vi "Get Local UTC Offset.vi"(9 "timestamp (now)":timestamp, 10 "UTC? (F)":bool) -> (1 "UTC Offset String":string, 2 "UTC Offset":T1=enum."UTC+00:00", 5 "UTC Offset (minutes)":i32, 7 "UTC Offset (hours)":i32)   [LabVIEW 2013]
uses:
  UTC Offsets -- enum.ctl
  <vilib>/regexp/Match Regular Expression.xnode
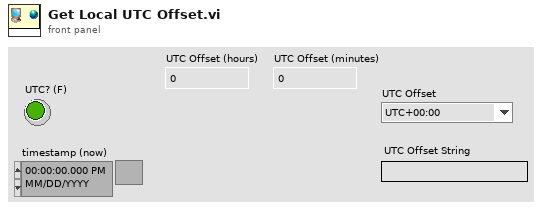
[diagram p1: front panel]
types:
  T1 = typedef "UTC Offsets -- enum.ctl" = enum16{"UTC-12:00", "UTC-11:00", "UTC-10:00", "UTC-09:30", "UTC-09:00", "UTC-08:00", "UTC-07:00", "UTC-06:00", "UTC-05:00", "UTC-04:00", "UTC-03:30", "UTC-03:00", "UTC-02:00", "UTC-01:00", "UTC-00:00", "UTC+00:00", "UTC+01:00", "UTC+02:00", "UTC+03:00", "UTC+03:30", "UTC+04:00", "UTC+04:30", "UTC+05:00", "UTC+05:30", "UTC+05:45", "UTC+06:00", "UTC+06:30", "UTC+07:00", "UTC+08:00", "UTC+08:45", "UTC+09:00", "UTC+09:30", "UTC+10:00", "UTC+10:30", "UTC+11:00", "UTC+12:00", "UTC+12:45", "UTC+13:00", "UTC+14:00"}
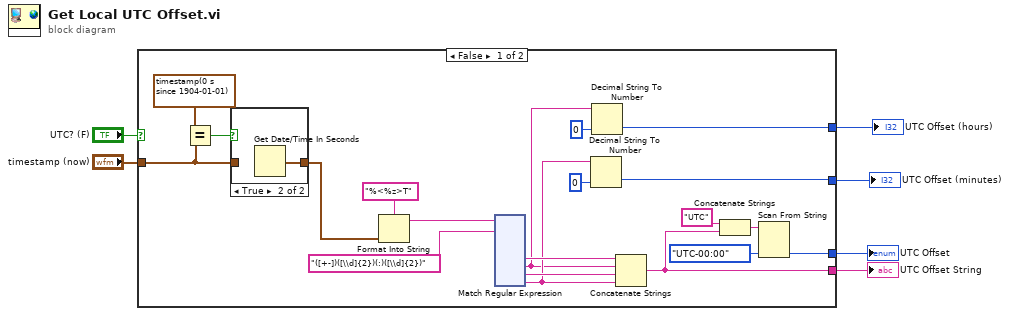
[diagram p0: block diagram]
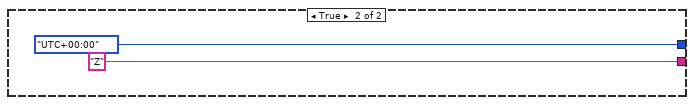
[diagram p3: hidden frame]
diagram:
  n1 = case shown="False" "UTC? (F)" {
    tunnel: [w26 UTC_Offsets_--_enum."UTC+00:00" ("UTC Time Offset")] -> w6
    tunnel: [w13 "Z"] -> w5
    tunnel: "timestamp (now)" -> [w20 _]
    tunnel: [w10 _] -> w2
    tunnel: [w7 _] -> w1
    frame False {
      n2 = Equal?(x=timestamp(0 s since 1904-01-01), y=w20) -> (x = y?=w22:bool)
      n3 = case shown="True" w22 {
        tunnel: [w146 w147] -> w18
        tunnel: w20 -> [w146 _]
        frame False {
        }
        frame True {
          n4 = Get Date/Time In Seconds() -> (seconds since 1Jan1904=w147:timestamp)
        }
      }
      n5 = Format Into String(format string="%<%z>T", w18) -> (resulting string=w17:string)  [unwired: 2 in, 1 out]
      n6 = xnode "Match Regular Expression"("input string"=w17, "regular expression"="([+-])([\\d]{2})(:)([\\d]{2})") -> ("submatch 1"=w15:string, "submatch 2"=w8:string, "submatch 3"=w14:string, "submatch 4"=w12:string)  [unwired: 4 in, 5 out]
      n7 = Decimal String To Number(string=w12, default (0L)=0 ("default (0 I32)")) -> (number=w10:i32)  [unwired: 1 in, 1 out]
      n8 = Decimal String To Number(string=w8, default (0L)=0 ("default (0 I32)")) -> (number=w7:i32)  [unwired: 1 in, 1 out]
      n9 = Concatenate Strings(w15, w8, w14, w12) -> (w13:string)
      n10 = Concatenate Strings("UTC" ("format string"), w13) -> (w24:string)
      n11 = Scan From String(input string=w24, default 1=UTC_Offsets_--_enum."UTC-00:00" ("UTC Time Offset")) -> (output 1=w26:T1)  [unwired: 3 in, 3 out]
    }
    frame True {
    }
  }
  "UTC Offset" <- w6
  "UTC Offset String" <- w5
  "UTC Offset (minutes)" <- w2
  "UTC Offset (hours)" <- w1
